vi "Test Resize.vi"() -> ()   [LabVIEW 2017, in "Image Processing Library.lvlib"]
uses:
  Image Processing Library.lvlib
panel:
  out "Image LetterBox Resize Cubic":picture
  out "Image LetterBox Resize":picture
  out "Image Resize":picture
  out "Image In":picture
  out "error out":errorcluster
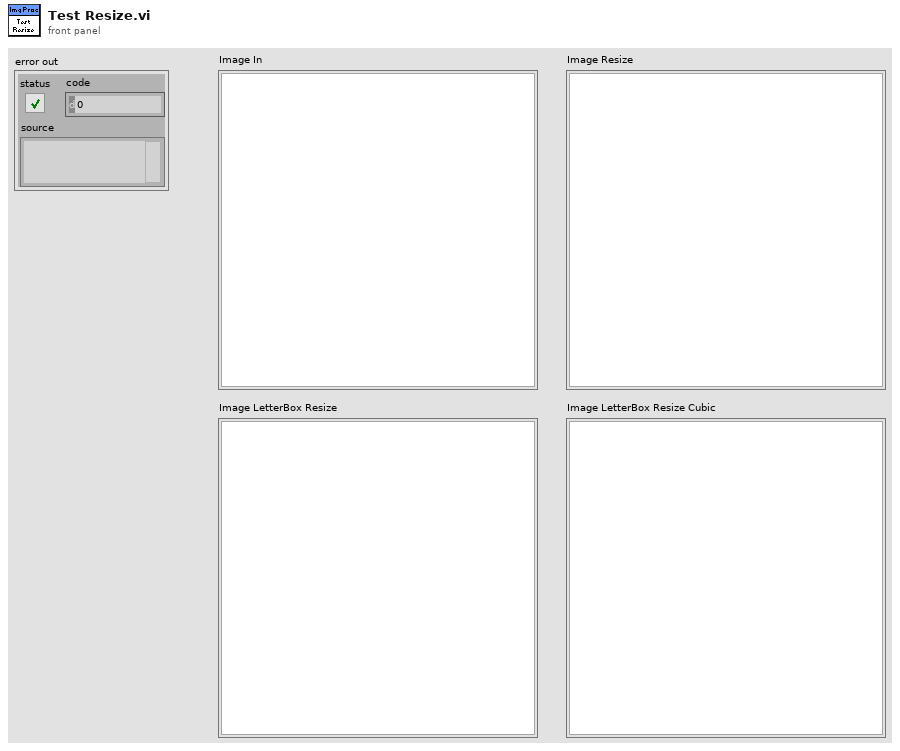
[diagram p1: front panel]
types:
  T1 = typedef "imagedata.ctl" = cluster{"image type":i32, "image depth":i32, "image":u8[], "mask":u8[], "colors":u32[], "Rectangle":cluster{"left":i16, "top":i16, "right":i16, "bottom":i16}}
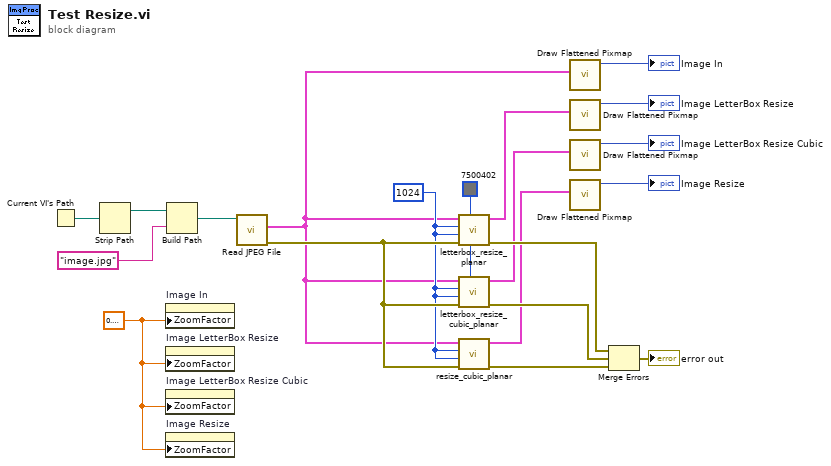
[diagram p0: block diagram]
diagram:
  w1 = sgl 0.3 ("Zoom Factor")
  w14 = 1024 ("target_w")
  w15 = u32 7500402 ("pad Color")
  n1 = Current VI's Path() -> (path=w19:path)
  n2 = Strip Path(path=w19) -> (stripped path=w18:path)  [unwired: 1 out]
  n3 = property on="Image In" class="Pict"("ZoomFactor"=w1) -> ()  [unwired: 2 in, 2 out]
  n4 = property on="Image LetterBox Resize" class="Pict"("ZoomFactor"=w1) -> ()  [unwired: 2 in, 2 out]
  n5 = property on="Image LetterBox Resize Cubic" class="Pict"("ZoomFactor"=w1) -> ()  [unwired: 2 in, 2 out]
  n6 = property on="Image Resize" class="Pict"("ZoomFactor"=w1) -> ()  [unwired: 2 in, 2 out]
  n7 = Build Path(base path=w18, name or relative path="image.jpg") -> (appended path=w17:path)
  n8 = call <vilib>:"Read JPEG File.vi"("path to JPEG file"=w17) -> ("error out"=w16:errorcluster, "image data"=w9:T1)  [unwired: 8 in, 1 out]
  n9 = call "letterbox_resize_planar.vi"("pad Color"=w15, "error in (no error)"=w16, "target_h"=w14, "target_w"=w14, "image in"=w9) -> ("error out"=w13:errorcluster, "image out"=w7:T1)  [unwired: 2 in, 3 out]
  n10 = call "letterbox_resize_cubic_planar.vi"("pad Color"=w15, "error in (no error)"=w16, "target_h"=w14, "target_w"=w14, "image in"=w9) -> ("error out"=w12:errorcluster, "image out"=w3:T1)  [unwired: 2 in, 3 out]
  n11 = call "resize_cubic_planar.vi"("error in (no error)"=w16, "target_h"=w14, "target_w"=w14, "image in"=w9) -> ("error out"=w11:errorcluster, "image out"=w2:T1)  [unwired: 6 in]
  n12 = call <vilib>:"Draw Flattened Pixmap.vi"("image data"=w9) -> ("new picture"=→"Image In":picture)  [unwired: 8 in]
  n13 = call <vilib>:"Draw Flattened Pixmap.vi"("image data"=w7) -> ("new picture"=→"Image LetterBox Resize":picture)  [unwired: 8 in]
  n14 = call <vilib>:"Draw Flattened Pixmap.vi"("image data"=w3) -> ("new picture"=→"Image LetterBox Resize Cubic":picture)  [unwired: 8 in]
  n15 = call <vilib>:"Draw Flattened Pixmap.vi"("image data"=w2) -> ("new picture"=→"Image Resize":picture)  [unwired: 8 in]
  n16 = Merge Errors(w13, w12, w11) -> (→"error out":errorcluster)
